vi "Get VI Refs To Translate.vi"(8 "error in (no error)":errorcluster, 10 "Top Level VI":refnum<vi>, 11 "Expected VIs":path[](array[path])) -> (0 "error out":errorcluster, 2 "VIs":path[](array[path]), 3 "VI Ref's":refnum<vi>[](array[refnum]), 5 "VIs Relative Path":path[](array[path]))   [LabVIEW 2019, in "Language Selection.lvlib"]
doc: "Initializes the VI translation.\n\nThis function should be used at the beginning of the Main VI in your project.\n- - -\nCopyright (c) 2026, Merecs Engineering GmbH"
uses:
  Language Selection.lvlib
panel:
  out "DependencyPaths (Debug)":path[](array[path])
  # "Connector Pane"
  # "Locals"
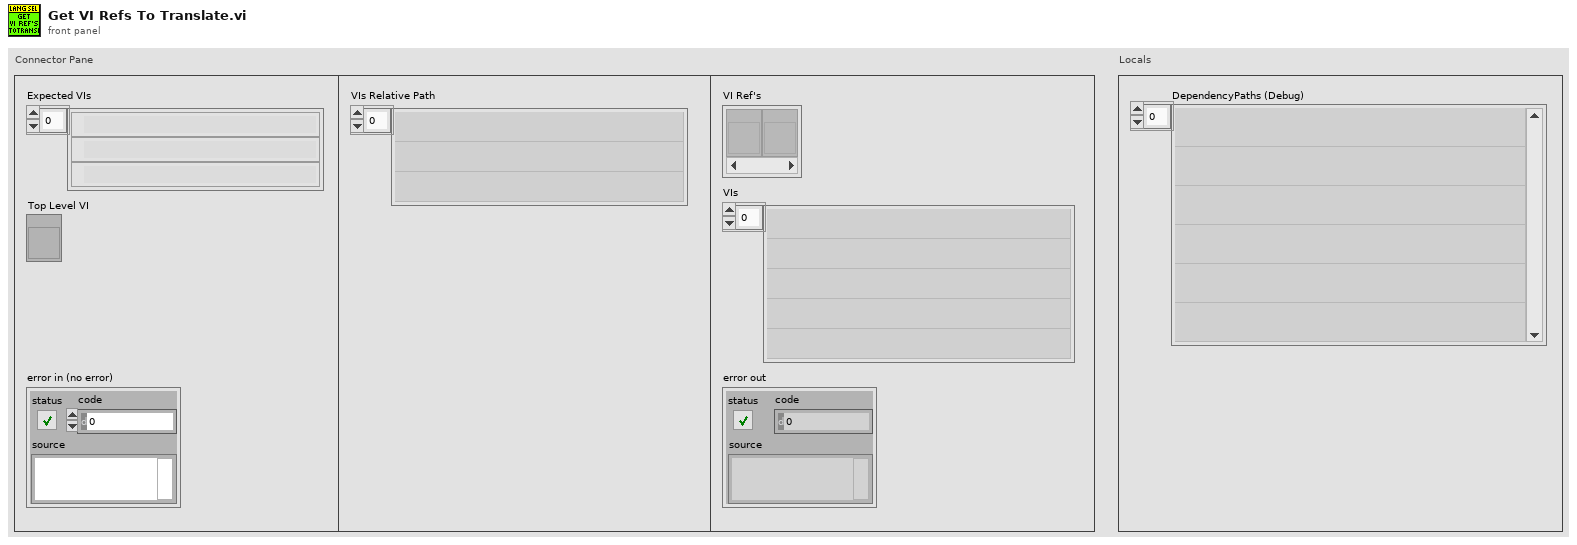
[diagram p1: front panel]
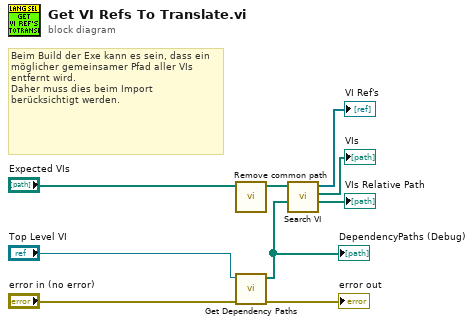
[diagram p0: block diagram]
diagram:
  # "Beim Build der Exe kann es sein, dass ein möglicher gemeinsamer Pfad aller VIs entfernt wird.\nDaher muss dies beim Import berücksichtigt werden."
  n1 = call "Remove common path.vi"("VI Paths In"="Expected VIs") -> ("VI Paths Out"=w1:path[])  [unwired: 10 in]
  n2 = call "Get Dependency Paths.vi"("error in (no error)"="error in (no error)", "VI in"="Top Level VI") -> ("error out"=→"error out":errorcluster, "DependencyPaths"=w7:path[])  [unwired: 8 in]
  "DependencyPaths (Debug)" <- w7
  n3 = call "Search VI.vi"("DependencyPaths"=w7, "Expected VIs"=w1) -> ("VIs Relative Path"=→"VIs Relative Path":path[], "VIs"=→"VIs":path[], "vi references"=→"VI Ref's":refnum<vi>[])  [unwired: 7 in]
